vi "range.vi"() -> ()   [LabVIEW 2025]
panel:
  out "Numeric":dbl
  in  "String":string
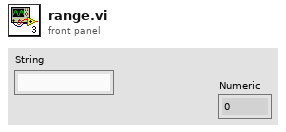
[diagram p1: front panel]
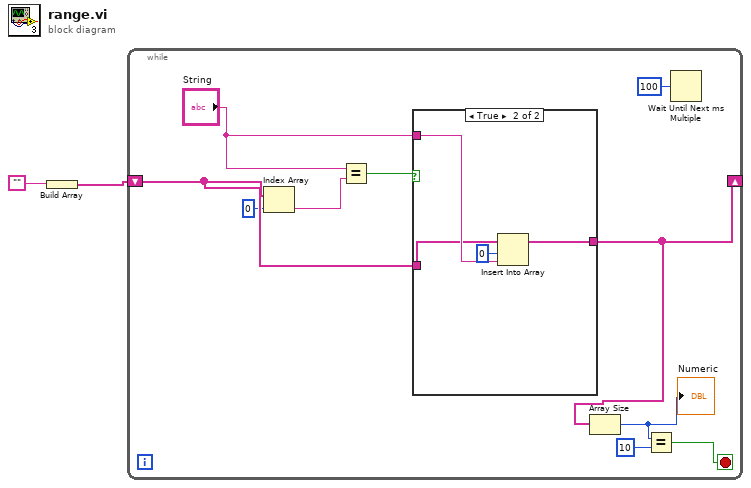
[diagram p0: block diagram]
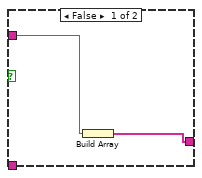
[diagram p2: hidden frame]
diagram:
  n1 = Build Array("") -> (w2:string[])
  n2 = while {
    shift-right: [w5] -> _
    shift-left: w2 -> [w10]
    stop <- w6 stop-if-true
    n3 = Index Array(array=w10, index=0) -> (element=w12:string)
    n4 = Equal?(x="String", y=w12) -> (x = y?=w11:bool)
    n5 = case shown="True" w11 {
      tunnel: w10 -> [_ w17]
      tunnel: "String" -> [w14 w18]
      tunnel: [w13 w15] -> w5
      frame False {
        n6 = Build Array(w14) -> (w13:string[])
      }
      frame True {
        n7 = Insert Into Array(array=w17, index=0, new element=w18) -> (w15:string[])
      }
    }
    n8 = Array Size(array=w5) -> (size(s)=w3:i32)
    "Numeric" <- w3
    n9 = Equal?(x=w3, y=10) -> (x = y?=w6:bool)
    n10 = Wait Until Next ms Multiple(millisecond multiple=u32 100) -> ()  [unwired: 1 out]
  }
